vi "Create String Channel.vi"(8 "error in (no error)":errorcluster, 10 "Channel Number":i32) -> (0 "error out":errorcluster, 2 "Boolean Channel":T1, 3 "Channel out":refnum<class "Channel.lvclass">)   [LabVIEW 2026, in "Modbus.lvlib" / "Modbus.lvclass"]
uses:
  Modbus.lvclass
  <vilib>/FlexLogger/SDK/PluginSDK.lvlibp/PEFClasses/SDK/Channel/Channel.lvclass
  Types/String Data.ctl
  Types/Modbus Table.ctl
  <vilib>/FlexLogger/SDK/PluginSDK.lvlibp/PEFClasses/SDK/Channel/Data Type_v2.ctl
  e0cdf0dc-ec87-4ce3-9d59-fa7e6132dbb7.vi
  <vilib>/FlexLogger/SDK/PluginSDK.lvlibp/PEFClasses/SDK/Producer Channel/Producer Channel.lvclass
  Globals/Modbus Strings.vi
  <vilib>/FlexLogger/SDK/PluginSDK.lvlibp/PEFClasses/SDK/Channel/ParameterAccess/Write I32.vi
  <vilib>/FlexLogger/SDK/PluginSDK.lvlibp/PEFClasses/SDK/Producer Channel/Create Producer Channel_v2.vi
  <vilib>/FlexLogger/SDK/PluginSDK.lvlibp/PEFClasses/SDK/Channel/ParameterAccess/Write Enum.vi
  <vilib>/FlexLogger/SDK/PluginSDK.lvlibp
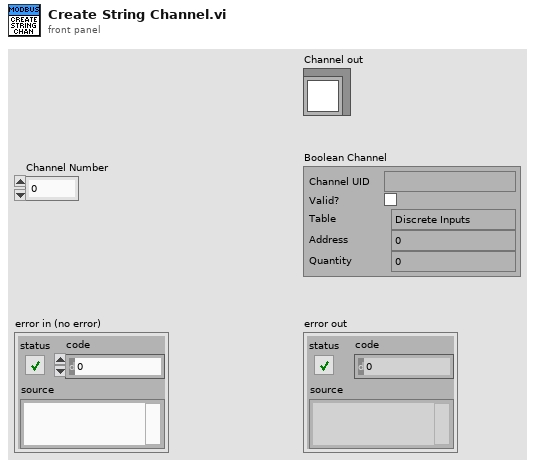
[diagram p1: front panel]
types:
  T1 = typedef "Modbus.lvlib/Modbus.lvclass/String Data.ctl" = cluster{"Channel UID":string, "Valid?":bool, "Table":T2, "Address":i32, "Quantity":u16}
  T2 = typedef "Modbus.lvlib/Modbus.lvclass/Modbus Table.ctl" = enum16{"Discrete Inputs", "Coils", "Input Registers", "Holding Registers"}
  T3 = typedef "PluginSDK.lvlibp/Channel.lvclass/Data Type_v2.ctl" = u16
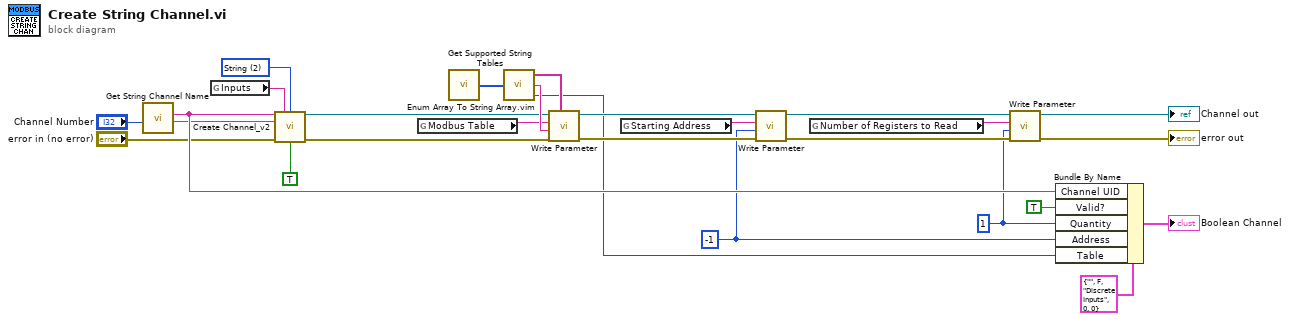
[diagram p0: block diagram]
diagram:
  w3 = u16 1 ("Value")
  w7 = T3 2 items=["Wfm (DBL)", "Wfm (Digital)", "String"] ("Data Type")
  w12 = -1 ("Value")
  n1 = call "Get String Channel Name.vi"("Channel Numer"="Channel Number") -> ("Bool Channel Name"=w8:string, "Bool Channel ID"=w27:string)  [unwired: 9 in]
  n2 = global read "Modbus Strings.vi" "Inputs"() -> (w10:string)
  n3 = call-poly <vilib>:"Create Channel_v2.vi"("Unique Channel Identifier"=w27, "Display Group"=w10, "Data Type"=w7, "Default Channel Name"=w8, "error in (no error)"="error in (no error)", "Can Disable?"=TRUE) -> ("Producer Channel"=w20:refnum<class "Producer Channel.lvclass">, "error out"=w21:errorcluster)  [unwired: 8 in]
  n4 = global read "Modbus Strings.vi" "Modbus Table"() -> (w18:string)
  n5 = call "Get Supported String Tables.vi"() -> ("Supported Tables"=w26:T2[])  [unwired: 1 in]
  n6 = call "Enum Array To String Array.vim"("Array of Enum Values"=w26) -> ("First Value"=w13:T2, "First String"=w23:string, "Strings out"=w22:string[])  [unwired: 2 in]
  n7 = call-poly <vilib>:"Write Parameter.vi"("Possible Values"=w22, "error in (no error)"=w21, "Current Value"=w23, "Name"=w18, "Channel in"=w20) -> ("error out"=w15:errorcluster, "Channel out"=w14:refnum<class "Producer Channel.lvclass">)  [unwired: 5 in]
  n8 = global read "Modbus Strings.vi" "Starting Address"() -> (w19:string)
  n9 = call-poly <vilib>:"Write Parameter.vi"("error in (no error)"=w15, "Value"=w12, "Name"=w19, "Channel in"=w14) -> ("error out"=w4:errorcluster, "Channel out"=w5:refnum<class "Producer Channel.lvclass">)  [unwired: 6 in]
  n10 = global read "Modbus Strings.vi" "Number of Registers to Read"() -> (w6:string)
  n11 = call-poly <vilib>:"Write Parameter.vi"("error in (no error)"=w4, "Value"=w3, "Name"=w6, "Channel in"=w5) -> ("error out"=→"error out":errorcluster, "Channel out"=→"Channel out":refnum<class "Producer Channel.lvclass">)  [unwired: 6 in]
  n12 = Bundle By Name(cluster=T1 {"Channel UID"="", "Valid?"=FALSE, "Table"=enum."Discrete Inputs", "Address"=0, "Quantity"=0} ("String Data"), "Channel UID"=w27, "Valid?"=TRUE, "Quantity"=w3, "Address"=w12, "Table"=w13) -> (→"Boolean Channel":T1)
